vi "ReadDataGet.vi"(7 "LabVIEW Web Service Request":refnum<class "Web Request.lvclass"> caption="LabVIEW 웹 서비스 요청") -> ()   [LabVIEW 2019]
uses:
  <vilib>/wsapi/Web Request.lvclass
  GlobalValue.vi
panel:
  # "웹 서비스 입력 터미널을 사용하여 웹 서비스 팔레트의 VI를 호출합니다. 팔레트에 접근하지 않아도 되는 경우를 제외하고는 커넥터 팬에서 제거하지 마십시오."
  # "커넥터 팬에 연결된 추가적인 컨트롤은 각각 URL의 입력으로 사용할 수 있습니다. 터미널 모드 출력에 인디케이터를 포함하려면(기본 설정), 역시 커넥터 팬에 연결되어야 합니다."
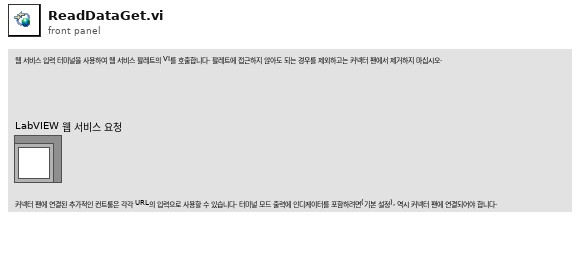
[diagram p1: front panel]
types:
  T1 = cluster{"Robot-M1509":cluster{"RobotState":dbl[], "Data":cluster{"Joint":cluster{"Position":dbl[], "Velocity":dbl[], "Current":dbl[], "Temperature":dbl[], "Torque":dbl[]}, "Task":cluster{"Position":dbl[], "Velocity":dbl[], "Euler":dbl[], "AngularVelocity":dbl[]}, "ExternalTCP":cluster{"Force":dbl[], "Moment":dbl[]}}}, "Robot-Delta":cluster{"Meta":cluster{"Timestamp":string, "Seq":dbl, "Model":string, "Online":string}, "Status":cluster{"ServoEnabled":string, "RobotMotion":string, "ErrorCode":string}, "Joint":cluster{"J13":cluster{"Position":dbl, "Speed":dbl, "Torque":dbl}, "J14":cluster{"Position":dbl, "Speed":dbl, "Torque":dbl}, "J15":cluster{"Position":dbl, "Speed":dbl, "Torque":dbl}}, "Cartesian":cluster{"X":dbl, "Y":dbl, "Z":dbl}}, "Robot_M1509":cluster{"Meta":cluster{"Timestamp":string, "Seq":dbl, "Model":string, "Online":string}, "Status":cluster{"RobotState":dbl[]}, "Joint":cluster{"J1":cluster{"Position":dbl, "Velocity":dbl, "Current":dbl, "Temperature":dbl, "Torque":dbl}, "J2":cluster{"Position":dbl, "Velocity":dbl, "Current":dbl, "Temperature":dbl, "Torque":dbl}, "J3":cluster{"Position":dbl, "Velocity":dbl, "Current":dbl, "Temperature":dbl, "Torque":dbl}, "J4":cluster{"Position":dbl, "Velocity":dbl, "Current":dbl, "Temperature":dbl, "Torque":dbl}, "J5":cluster{"Position":dbl, "Velocity":dbl, "Current":dbl, "Temperature":dbl, "Torque":dbl}, "J6":cluster{"Position":dbl, "Velocity":dbl, "Current":dbl, "Temperature":dbl, "Torque":dbl}}, "Cartesian":cluster{"Position":cluster{"X":dbl, "Y":dbl, "Z":dbl}, "Orientation":cluster{"Rx":dbl, "Ry":dbl, "Rz":dbl}, "Velocitiy":cluster{"X":dbl, "Y":dbl, "Z":dbl}, "Augularvelocity":cluster{"Rx":dbl, "Ry":dbl, "Rz":dbl}}, "ExternalTCP":cluster{"Force":cluster{"X":dbl, "Y":dbl, "Z":dbl}, "Moment":cluster{"Rx":dbl, "Ry":dbl, "Rz":dbl}}}, "Robot-HH7":cluster{"Meta":cluster{"Timestamp":string, "Model":string, "Online":string, "Seq":dbl}, "Status":cluster{"RobotMode":dbl, "Playback":dbl, "RemoteMode":dbl}, "Joint":cluster{"J1":cluster{"Position":dbl, "Velocity":dbl, "Current":dbl, "Temperature":dbl, "Torque":dbl}, "J2":cluster{"Position":dbl, "Velocity":dbl, "Current":dbl, "Temperature":dbl, "Torque":dbl}, "J3":cluster{"Position":dbl, "Velocity":dbl, "Current":dbl, "Temperature":dbl, "Torque":dbl}, "J4":cluster{"Position":dbl, "Velocity":dbl, "Current":dbl, "Temperature":dbl, "Torque":dbl}, "J5":cluster{"Position":dbl, "Velocity":dbl, "Current":dbl, "Temperature":dbl, "Torque":dbl}, "J6":cluster{"Position":dbl, "Velocity":dbl, "Current":dbl, "Temperature":dbl, "Torque":dbl}}, "Cartesian":cluster{"Position":cluster{"X":dbl, "Y":dbl, "Z":dbl}, "Orientation":cluster{"Rx":dbl, "Ry":dbl, "Rz":dbl}, "Velocitiy":cluster{"X":dbl, "Y":dbl, "Z":dbl}, "Augularvelocity":cluster{"Rx":dbl, "Ry":dbl, "Rz":dbl}}, "ExternalTCP":cluster{"Force":cluster{"X":dbl, "Y":dbl, "Z":dbl}, "Moment":cluster{"Rx":dbl, "Ry":dbl, "Rz":dbl}}}, "Robot-AMR":cluster{"Meta":cluster{"Timestamp":string, "Model":string, "Seq":dbl, "Online":bool}, "LastUpdate":cluster{"Pose":string, "Speed":string, "BaseEncode":string}, "Status":cluster{"NavStatus":dbl, "EmergencyButton":dbl, "ChargeFlag":dbl}, "Pose":cluster{"X":dbl, "Y":dbl, "Theta":dbl}, "Speed":cluster{"Vx":dbl, "Vth":dbl}, "Battery":cluster{"Level":dbl}, "Errors":cluster{"NavStatus":string}}}
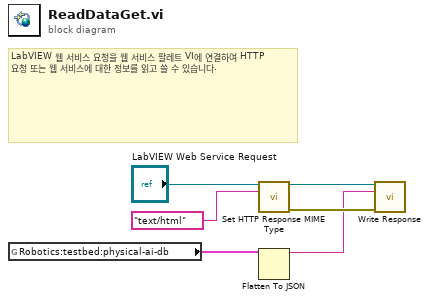
[diagram p0: block diagram]
diagram:
  # "LabVIEW 웹 서비스 요청을 웹 서비스 팔레트 VI에 연결하여 HTTP 요청 또는 웹 서비스에 대한 정보를 읽고 쓸 수 있습니다."
  n1 = global read "GlobalValue.vi" "Robotics:testbed:physical-ai-db"() -> (w1:T1)
  n2 = call <vilib>:"Set HTTP Response MIME Type.vi"("LabVIEW Web Service Request"="LabVIEW Web Service Request", "MIME type (text/html)"="text/html") -> ("LabVIEW Web Service Request out"=w5:refnum<class "Web Request.lvclass">, "error out"=w3:errorcluster)  [unwired: 12 in]
  n3 = Flatten To JSON(anything=w1) -> (JSON string=w2:string)  [unwired: 2 in, 1 out]
  n4 = call <vilib>:"Write Response.vi"("LabVIEW Web Service Request"=w5, "response string"=w2, "error in (no error)"=w3) -> ()  [unwired: 11 in, 2 out]
